vi "DAQ_Test.vi"() -> ()   [LabVIEW 2025]
uses:
  <vilib>/measure/NI_MAPro.lvlib
panel:
  out "DC value":dbl format="%0.2p"
  out "RMS value":dbl format="%0.2p"
  out "data":dynamicdata(graph)
  in  "stop (F)":bool
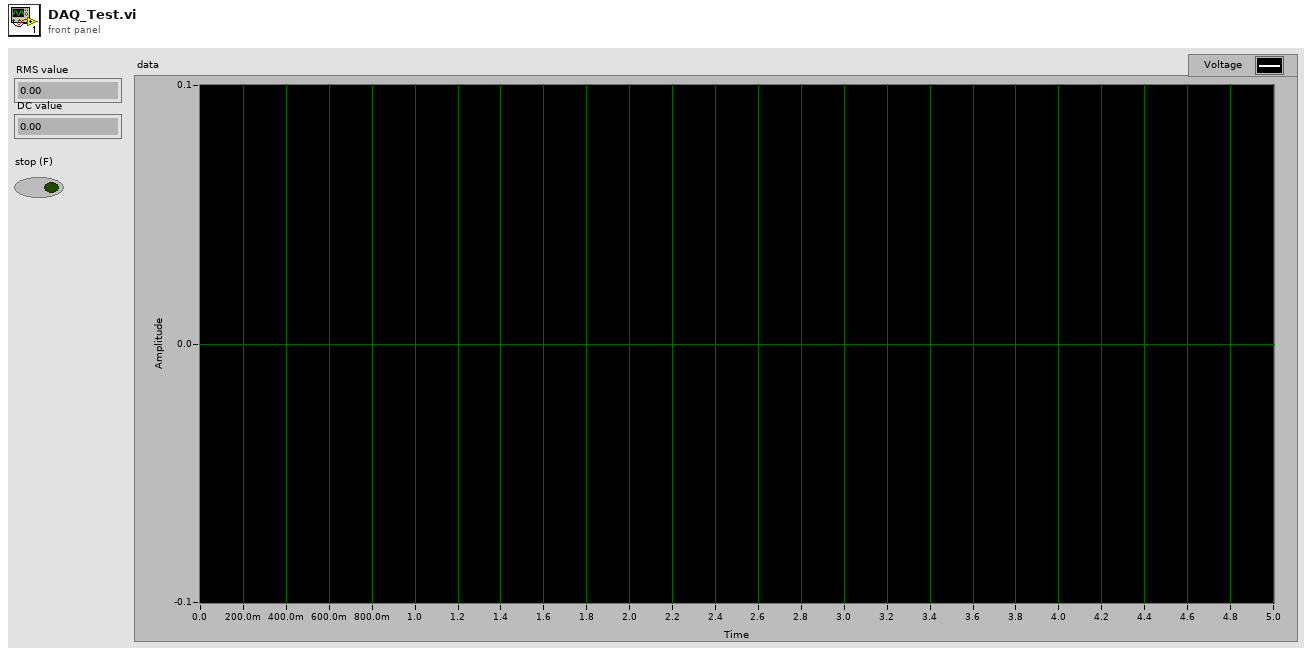
[diagram p1: front panel]
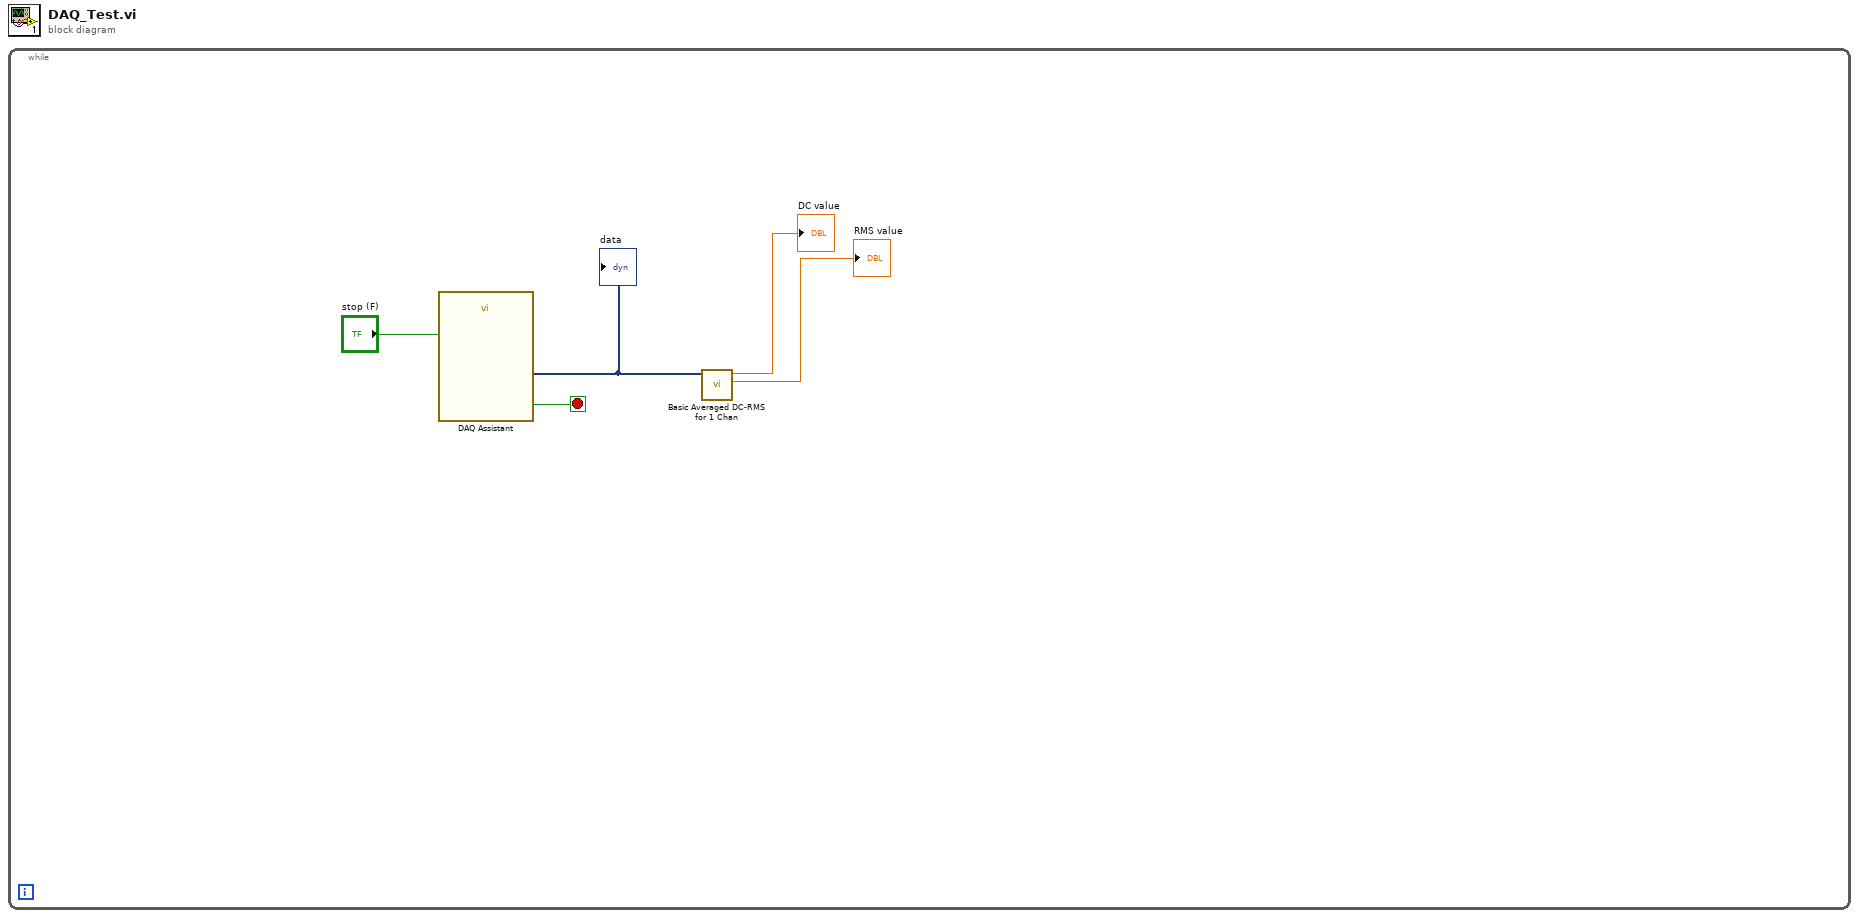
[diagram p0: block diagram]
diagram:
  n1 = while {
    stop <- w4 stop-if-true
    n2 = call "DAQ Assistant"("stop (F)"="stop (F)") -> ("data"=w3:dynamicdata, "stopped"=w4:bool)  [unwired: 15 in, 2 out]
    "data" <- w3
    n3 = call <vilib>:"Basic Averaged DC-RMS for 1 Chan.vi"("signal in"=w3) -> ("RMS value"=→"RMS value":dbl, "DC value"=→"DC value":dbl)  [unwired: 7 in, 2 out]
  }
